vi "TC10 Update.vi"(5 "TC10 State LED ref":refnum<vi>, 7 "INTERFACE NAME ref":refnum<vi>, 8 "error in":errorcluster, 11 "XNET Session in":refnum<k21>) -> (0 "error out":errorcluster, 3 "XNET Session out":refnum<k21>)   [LabVIEW 2025, in "Automotive Ethernet Bus Monitor UI.lvlib"]
doc: "Update the TC10 session and state LED."
uses:
  Automotive Ethernet Bus Monitor UI.lvlib
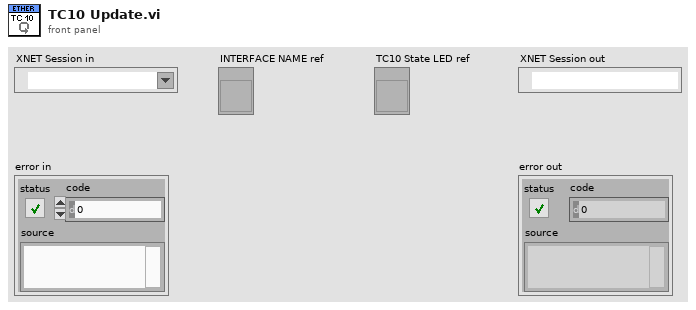
[diagram p1: front panel]
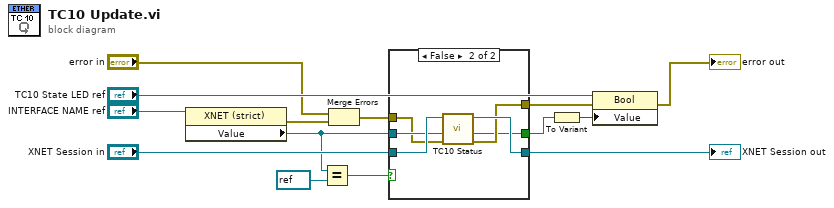
[diagram p0: block diagram]
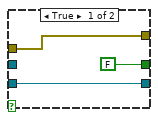
[diagram p2: hidden frame]
diagram:
  n1 = property class="XNET (strict)"(reference="INTERFACE NAME ref") -> (error out=w7:errorcluster, "Value"=w2:refnum<k21>)  [unwired: 1 in, 1 out]
  n2 = Equal?(x=w2, y=refnum<k21> refnum) -> (x = y?=w3:bool)
  n3 = Merge Errors("error in", w7) -> (w5:errorcluster)
  n4 = case shown="False" w3 {
    tunnel: [FALSE ("TC10 Mode") w18] -> w12
    tunnel: "XNET Session in" -> [w15 w23]
    tunnel: [w15 w22] -> w11
    tunnel: w2 -> [_ w21]
    tunnel: [w17 w20] -> w10
    tunnel: w5 -> [w17 w19]
    frame True {
    }
    frame False {
      n5 = call "TC10 Status.vi"("error in (no error)"=w19, "Interface Name"=w21, "XNET Session"=w23) -> ("error out"=w20:errorcluster, "TC10 Mode"=w18:bool, "XNET Session Out"=w22:refnum<k21>)  [unwired: 6 in]
    }
  }
  "XNET Session out" <- w11
  n6 = To Variant(anything=w12) -> (Variant=w13:variant)
  n7 = property class="Bool"(reference="TC10 State LED ref", error in=w10, "Value"=w13) -> (error out=→"error out":errorcluster)  [unwired: 1 out]
